vi "Replace Line.vi"(8 "error in":errorcluster, 9 "New Line":T1, 10 "Line Name":string, 11 "Scan Engine configuration in":refnum<class "Scan Engine configuration.lvclass">) -> (0 "error out":errorcluster, 2 "Old Line":T1, 3 "Scan Engine configuration out":refnum<class "Scan Engine configuration.lvclass">)   [LabVIEW 2015, in "Scan Engine configuration.lvclass"]
uses:
  Scan Engine configuration.lvclass
  Line.ctl
  <vilib>/NI/Tag Bus Module Framework/channel/TBM channel.lvclass
  Scan Engine configuration.lvclass/Scan Engine configuration.ctl
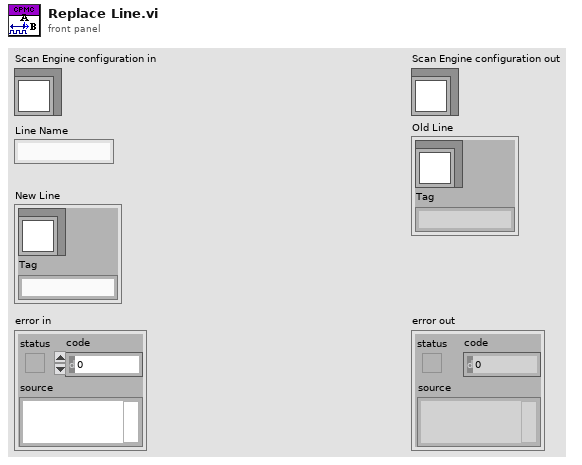
[diagram p1: front panel]
types:
  T1 = typedef "Scan Engine configuration.lvclass/Line.ctl" = cluster{"channel":refnum<class "TBM channel.lvclass">, "Tag":string}
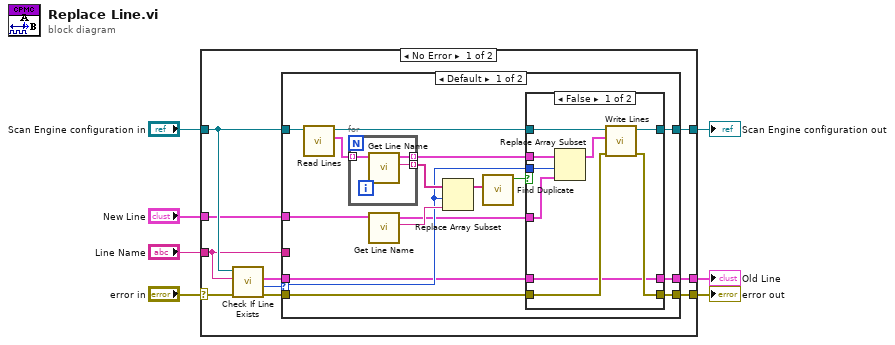
[diagram p0: block diagram]
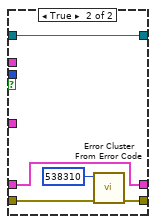
[diagram p2: hidden frame]
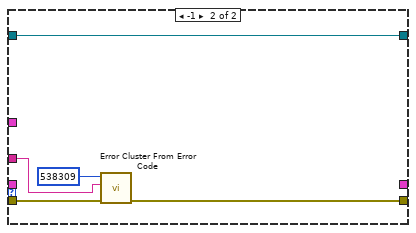
[diagram p3: hidden frame]
diagram:
  n1 = case shown="No Error" "error in" {
    selector: "error in" -> [w10 w57]
    tunnel: [w16 w57] -> w6
    tunnel: [w17 w56] -> w4
    tunnel: "Scan Engine configuration in" -> [w15 w56]
    tunnel: "Line Name" -> [w14 _]
    tunnel: "New Line" -> [w12 _]
    tunnel: [w11 _] -> w1
    frame No Error {
      n2 = call-dynamic "Check If Line Exists.vi"("error in"=w10, "name to locate"=w14, "Scan Engine configuration in"=w15) -> ("error out"=w9:errorcluster, "index"=w13:i32, "Line out"=w8:T1)  [unwired: 4 in, 2 out]
      n3 = case shown="Default" w13 {
        selector: w13 -> [w25 _]
        tunnel: w15 -> [w32 w55]
        tunnel: [w33 w55] -> w17
        tunnel: w12 -> [w29 _]
        tunnel: w14 -> [_ w51]
        tunnel: w9 -> [w21 w53]
        tunnel: [w20 w52] -> w16
        tunnel: [w19 _] -> w11
        tunnel: w8 -> [w18 _]
        frame Default {
          n4 = call "Read Lines.vi"("Scan Engine configuration in"=w32) -> ("Lines"=w30:T1[], "Scan Engine configuration out"=w31:refnum<class "Scan Engine configuration.lvclass">)  [unwired: 8 in, 1 out]
          n5 = for {
            tunnel: w30 -> [w50] mode=indexing
            tunnel: [w49] -> w26 mode=indexing
            tunnel: [w48] -> w28 mode=indexing
            n6 = call "Get Line Name.vi"("Line in"=w50) -> ("Name"=w48:string, "Line out"=w49:T1)  [unwired: 8 in, 1 out]
          }
          n7 = call "Get Line Name.vi"("Line in"=w29) -> ("Name"=w27:string, "Line out"=w24:T1)  [unwired: 8 in, 1 out]
          n8 = Replace Array Subset(array=w28, new element=w27, index=w25) -> (w23:string[])
          n9 = call "Find Duplicate.vi"("Array"=w23) -> ("Duplicate"=w22:bool)  [unwired: 8 in, 2 out]
          n10 = case shown="False" w22 {
            tunnel: [w37 w44] -> w33
            tunnel: w31 -> [w39 w44]
            tunnel: w26 -> [w42 _]
            tunnel: w25 -> [w41 _]
            tunnel: w24 -> [w40 _]
            tunnel: w21 -> [w36 w47]
            tunnel: [w35 w46] -> w20
            tunnel: [w34 w45] -> w19
            tunnel: w18 -> [w34 w45]
            frame False {
              n11 = Replace Array Subset(array=w42, new element=w40, index=w41) -> (w38:T1[])
              n12 = call "Write Lines.vi"("error in (no error)"=w36, "Lines"=w38, "Scan Engine configuration in"=w39) -> ("error out"=w35:errorcluster, "Scan Engine configuration out"=w37:refnum<class "Scan Engine configuration.lvclass">)  [unwired: 7 in]
            }
            frame True {
              n13 = call <vilib>:"Error Cluster From Error Code.vi"("error in (no error)"=w47, "error code (0)"=538310) -> ("error out"=w46:errorcluster)  [unwired: 7 in]
            }
          }
        }
        frame -1 {
          n14 = call <vilib>:"Error Cluster From Error Code.vi"("error in (no error)"=w53, "error message (\"\")"=w51, "error code (0)"=538309) -> ("error out"=w52:errorcluster)  [unwired: 6 in]
        }
      }
    }
    frame Error {
    }
  }
  "error out" <- w6
  "Scan Engine configuration out" <- w4
  "Old Line" <- w1
